vi "BNAL Csave Preaparation VI.vi"(6 "BNAL TD":T1, 7 "SB_ANA":T3, 8 "error in":errorcluster caption="エラー入力", 9 "Total assembly C":T4 {"Assembly Ratio 2" format="%#_3g"; "Assembly Ratio" format="%#_3g"}, 10 "B prep":T2, 11 "TDMSファイル in":refnum<k34>) -> (0 "error out":errorcluster, 3 "file path out":path)   [LabVIEW 2018]
panel:
  out "転置配列":string[][](array[string])
  out "BR Table Data":string[](array[string])
  out "BR Table Tag":string[](array[string])
  out "BNAL updata Date":string
  out "BNAL Program version":string
  out "Base Cutted Q#":i32
  out "RRS#":i32
  out "all option#":i32
  out "RR option#":i32
  out "Base Species#":i32
  out "RR Ratio (%)":dbl
  out "Assembly Ratio 2":dbl
  out "Signal #":i32
  out "Long Signal#":i32
  out "Assembly Ratio":dbl
  out "Av R_Read N":dbl format="%#_4g"
  out "Av N_Read N":dbl format="%#_4g"
  out "coverage [%]":dbl format="%#.2g"
  out "5’→3'":dbl format="%#.3g"
  out "Total Base CP":i32
  out "RR MIN Over S#":i32
  out "Av n#bp":i32
  out "Av RR n#bp":i32
  out "Av RRn# kbp/day":dbl format="%#_3f"
  out "Av n# kbp/day":dbl format="%#_3f"
  out "RR#":i32
  out "S#":i32
  out "Covered?":bool
  out "MAX RR#":i32
  out "Bnal Time":string
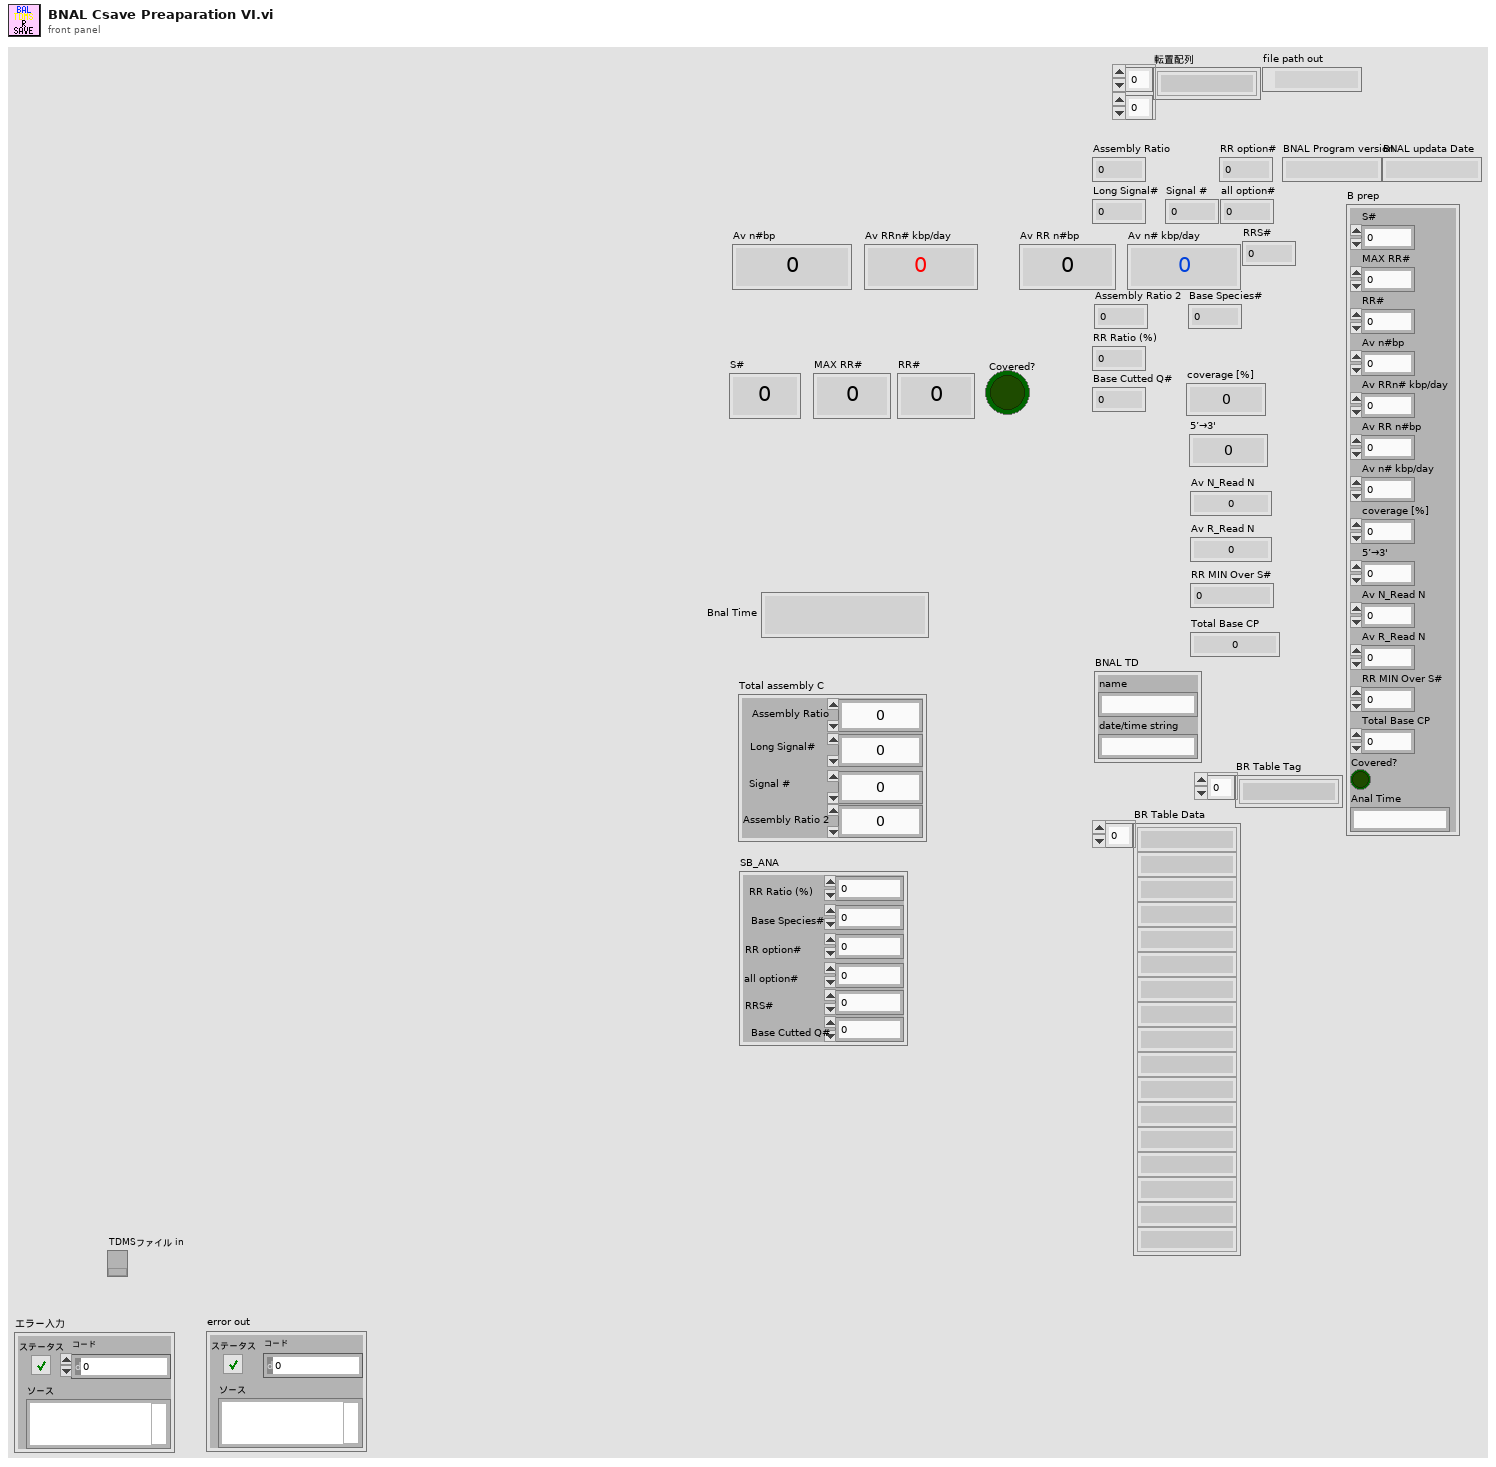
[diagram p1: front panel]
types:
  T1 = cluster{"name":string, "date/time string":string}
  T2 = cluster{"S#":i32, "MAX RR#":i32, "RR#":i32, "Av n#bp":i32, "Av RRn# kbp/day":dbl, "Av RR n#bp":i32, "Av n# kbp/day":dbl, "coverage [%]":dbl, "5’→3'":dbl, "Av N_Read N":dbl, "Av R_Read N":dbl, "RR MIN Over S#":i32, "Total Base CP":i32, "Covered?":bool, "Anal Time":string}
  T3 = cluster{"RR Ratio (%)":dbl, "Base Species#":i32, "RR option#":i32, "all option#":i32, "RRS#":i32, "Base Cutted Q#":i32}
  T4 = cluster{"Assembly Ratio":dbl, "Long Signal#":i32, "Signal #":i32, "Assembly Ratio 2":dbl}
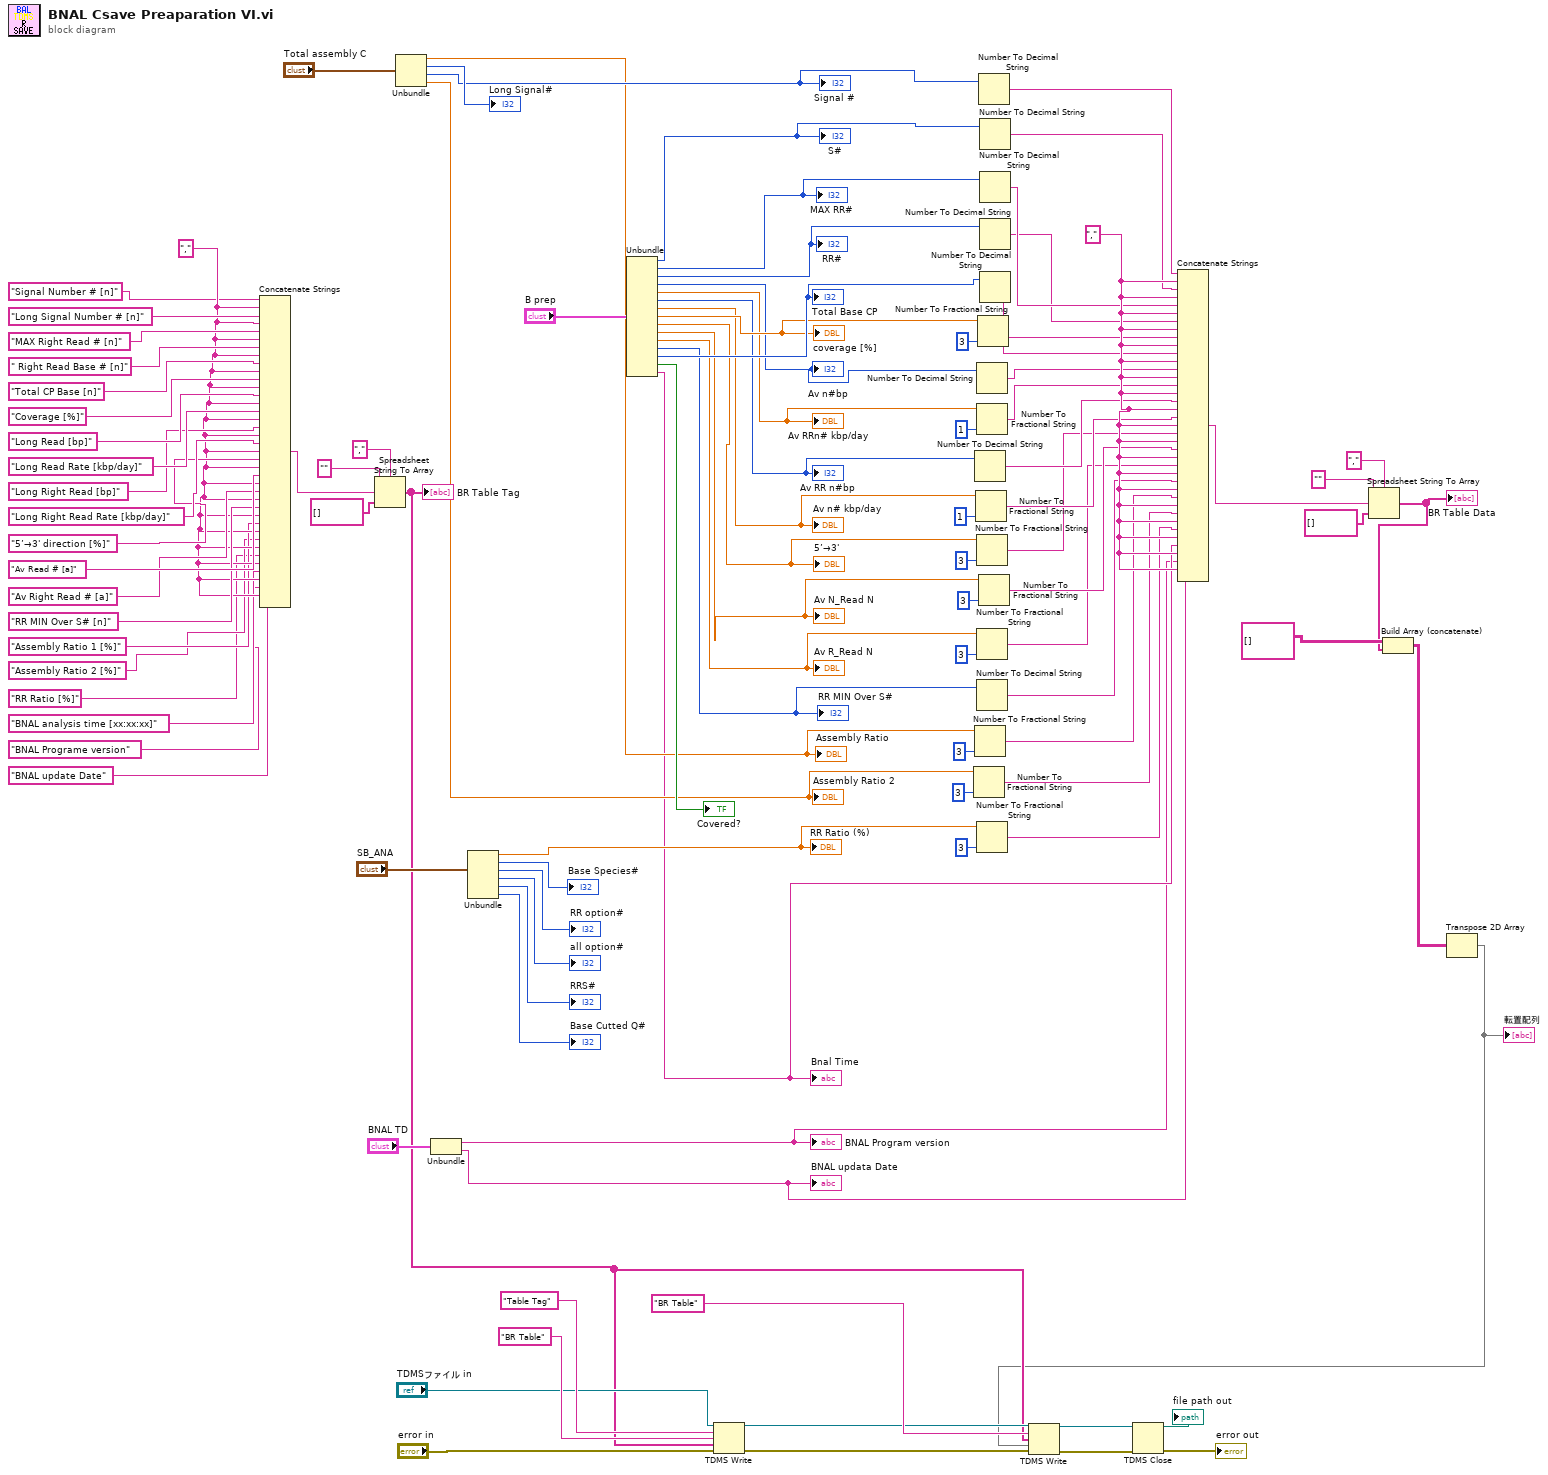
[diagram p0: block diagram]
diagram:
  w71 = ","
  w79 = ","
  n1 = Concatenate Strings("Signal Number # [n]", w79, "Long Signal Number # [n]", w79, "MAX Right Read # [n]", w79, " Right Read Base # [n]", w79, "Total CP Base [n]", w79, "Coverage [%]", w79, "Long Read [bp]", w79, "Long Read Rate [kbp/day]", w79, "Long Right Read [bp]", w79, "Long Right Read Rate [kbp/day]", w79, "5’→3' direction [%]", w79, "Av Read # [a]", w79, "Av Right Read # [a]", w79, "RR MIN Over S# [n]", w79, "Assembly Ratio 1 [%]", w79, "Assembly Ratio 2 [%]", w79, "RR Ratio [%]", w79, "BNAL analysis time [xx:xx:xx]", w79, "BNAL Programe version", w79, "BNAL update Date") -> (w21:string)
  n2 = Spreadsheet String To Array(delimiter (Tab)="," ("デリミタ（タブ）"), format string="" ("形式文字列"), spreadsheet string=w21, array type (2D Dbl)=string[] [] ("行ヘッダ文字列[]")) -> (array=w6:string[])
  "BR Table Tag" <- w6
  n3 = Unbundle("Total assembly C") -> ("Assembly Ratio"=w33:dbl, "Long Signal#"=→"Long Signal#":i32, "Signal #"=w70:i32, "Assembly Ratio 2"=w32:dbl)
  "Assembly Ratio" <- w33
  "Signal #" <- w70
  "Assembly Ratio 2" <- w32
  n4 = Unbundle("BNAL TD") -> ("name"=w26:string, "date/time string"=w25:string)
  "BNAL Program version" <- w26
  "BNAL updata Date" <- w25
  n5 = Unbundle("SB_ANA") -> ("RR Ratio (%)"=w31:dbl, "Base Species#"=→"Base Species#":i32, "RR option#"=→"RR option#":i32, "all option#"=→"all option#":i32, "RRS#"=→"RRS#":i32, "Base Cutted Q#"=→"Base Cutted Q#":i32)
  "RR Ratio (%)" <- w31
  n6 = Unbundle("B prep") -> ("S#"=w68:i32, "MAX RR#"=w66:i32, "RR#"=w62:i32, "Av n#bp"=w57:i32, "Av RRn# kbp/day"=w54:dbl, "Av RR n#bp"=w52:i32, "Av n# kbp/day"=w49:dbl, "coverage [%]"=w59:dbl, "5’→3'"=w46:dbl, "Av N_Read N"=w42:dbl, "Av R_Read N"=w41:dbl, "RR MIN Over S#"=w38:i32, "Total Base CP"=w61:i32, "Covered?"=→"Covered?":bool, "Anal Time"=w27:string)
  "Bnal Time" <- w27
  "MAX RR#" <- w66
  "S#" <- w68
  "RR#" <- w62
  "Av n# kbp/day" <- w49
  "Av RRn# kbp/day" <- w54
  "Av RR n#bp" <- w52
  "Av n#bp" <- w57
  "RR MIN Over S#" <- w38
  "Total Base CP" <- w61
  "5’→3'" <- w46
  "coverage [%]" <- w59
  "Av N_Read N" <- w42
  "Av R_Read N" <- w41
  n7 = TDMS Write(0:"TDMSファイル in", 5:"Table Tag" ("グループ名入力（名称未設定）"), 7:"BR Table" ("Group name"), 9:w6, 11:"error in") -> (4:w11:refnum<k34>, 15:w12:errorcluster)  [unwired: 1 in, 2 out]
  n8 = Number To Fractional String(number=w32, precision (6)=i16 3 ("精度（6）")) -> (F-format string=w29:string)  [unwired: 2 in]
  n9 = Number To Decimal String(number=w52) -> (decimal integer string=w51:string)  [unwired: 1 in]
  n10 = Number To Fractional String(number=w33, precision (6)=i16 3 ("精度（6）")) -> (F-format string=w30:string)  [unwired: 2 in]
  n11 = Number To Fractional String(number=w49, precision (6)=i16 1 ("精度（6）")) -> (F-format string=w48:string)  [unwired: 2 in]
  n12 = Number To Decimal String(number=w57) -> (decimal integer string=w56:string)  [unwired: 1 in]
  n13 = Number To Fractional String(number=w54, precision (6)=i16 1 ("精度（6）")) -> (F-format string=w53:string)  [unwired: 2 in]
  n14 = Number To Fractional String(number=w46, precision (6)=i16 3 ("精度（6）")) -> (F-format string=w45:string)  [unwired: 2 in]
  n15 = Number To Fractional String(number=w41, precision (6)=i16 3 ("精度（6）")) -> (F-format string=w39:string)  [unwired: 2 in]
  n16 = Number To Decimal String(number=w38) -> (decimal integer string=w37:string)  [unwired: 1 in]
  n17 = Number To Fractional String(number=w31, precision (6)=i16 3 ("精度（6）")) -> (F-format string=w28:string)  [unwired: 2 in]
  n18 = Number To Fractional String(number=w59, precision (6)=i16 3 ("精度（6）")) -> (F-format string=w58:string)  [unwired: 2 in]
  n19 = Number To Decimal String(number=w70) -> (decimal integer string=w69:string)  [unwired: 1 in]
  n20 = Number To Fractional String(number=w42, precision (6)=i16 3 ("精度（6）")) -> (F-format string=w40:string)  [unwired: 2 in]
  n21 = Number To Decimal String(number=w68) -> (decimal integer string=w67:string)  [unwired: 1 in]
  n22 = Number To Decimal String(number=w66) -> (decimal integer string=w65:string)  [unwired: 1 in]
  n23 = Number To Decimal String(number=w62) -> (decimal integer string=w64:string)  [unwired: 1 in]
  n24 = Number To Decimal String(number=w61) -> (decimal integer string=w63:string)  [unwired: 1 in]
  n25 = Concatenate Strings(w69, w71, w67, w71, w65, w71, w64, w71, w63, w71, w58, w71, w56, w71, w53, w71, w51, w71, w48, w71, w45, w71, w40, w71, w39, w71, w37, w71, w30, w71, w29, w71, w28, w71, w27, w71, w26, w71, w25) -> (w17:string)
  n26 = Spreadsheet String To Array(delimiter (Tab)="," ("デリミタ（タブ）"), format string="" ("形式文字列"), spreadsheet string=w17, array type (2D Dbl)=string[] [] ("行ヘッダ文字列[]")) -> (array=w14:string[])
  "BR Table Data" <- w14
  n27 = Build Array (concatenate)(string[][] [] ("Table"), w14) -> (w15:string[][])
  n28 = Transpose 2D Array(2D array=w15) -> (transposed array=w5:string[][])
  "転置配列" <- w5
  n29 = TDMS Write(0:w11, 5:"BR Table" ("Group name"), 7:w6, 9:w5, 11:w12) -> (4:w2:refnum<k34>, 15:w4:errorcluster)  [unwired: 1 in, 2 out]
  n30 = TDMS Close(8:w4, 11:w2) -> (0:→"error out":errorcluster, 3:→"file path out":path)
